vi "linked-ignore.vi"(0 "Ignored command":string="echo fixture-only-one", 5 "Reported command":string="echo fixture-only-two", 11 "error in":errorcluster) -> (15 "error out":errorcluster)   [LabVIEW 2024]
doc: "Static analysis fixture with two System Exec calls and an ignore arrow on only the first call. Do not run this VI: execution would launch external commands."
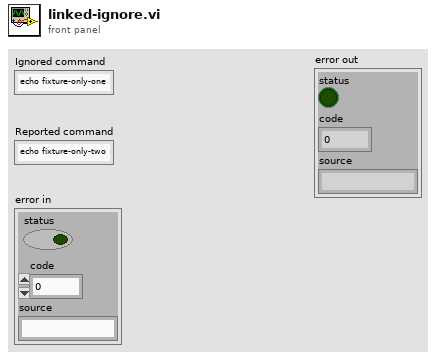
[diagram p1: front panel]
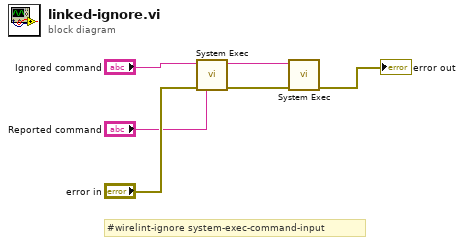
[diagram p0: block diagram]
diagram:
  # "#wirelint-ignore system-exec-command-input"
  n1 = call <vilib>:"System Exec.vi"("error in (no error)"="error in", "command line"="Ignored command") -> ("error out"=w4:errorcluster)  [unwired: 6 in, 3 out]
  n2 = call <vilib>:"System Exec.vi"("error in (no error)"=w4, "command line"="Reported command") -> ("error out"=→"error out":errorcluster)  [unwired: 6 in, 3 out]
